vi "VIH Utility - STR - Constant String To Array.vi"(11 "String in":string) -> (3 "Array out":string[](array[string]))   [LabVIEW 2014]
doc: "::: VI Helpeks :::\nCopyright (c) 2000-2026 Konstantin Shifershteyn. All rights reserved."
panel:
  # "VI Helpeks\nCopyright (c) 2012-2026 Konstantin Shifershteyn"
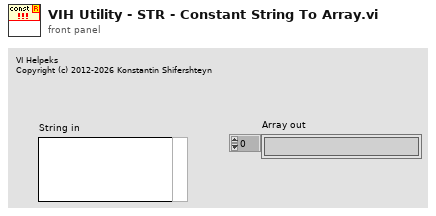
[diagram p1: front panel]
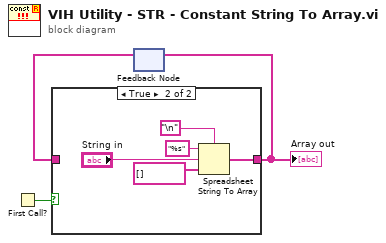
[diagram p0: block diagram]
diagram:
  n1 = First Call?() -> (First Call?: T/F=w1:bool)
  n2 = feedback #1() -> (w2:string[])  [unwired: 1 in]
  n3 = case shown="True" w1 {
    tunnel: [w4 w9] -> w3
    tunnel: w2 -> [w4 _]
    frame False {
    }
    frame True {
      n4 = Spreadsheet String To Array(delimiter (Tab)="\n" ("delimiter ('\\n')"), format string="%s", spreadsheet string="String in", array type (2D Dbl)=string[] [] ("Array out")) -> (array=w9:string[])
    }
  }
  "Array out" <- w3
  n5 = feedback-in #1(w3) -> ()
